vi "Test MQTT-3.1.2-12.vi"(8 "error in (no error)":errorcluster) -> (0 "error out":errorcluster)   [LabVIEW 2013]
uses:
  <vilib>/LabVIEW Open Source Project/MQTT Control Packets/Control Packets/ControlPacket/ControlPacket.lvclass
  <vilib>/LabVIEW Open Source Project/MQTT Control Packets/Control Packets/CONNECT/ConnectFlags -- cluster.ctl
  <vilib>/LabVIEW Open Source Project/MQTT Control Packets/Control Packets/ControlPacket/QualityOfService -- enum.ctl
  <vilib>/LabVIEW Open Source Project/MQTT Client/Client class/Client.lvclass/Client.ctl
  <vilib>/addons/_JKI Toolkits/Caraya/classes/Assert/Assert Equal Value_Variant.vi
  <vilib>/addons/_JKI Toolkits/Caraya/classes/Assert/Assert Equal Value and Type_Variant.vi
  <vilib>/LabVIEW Open Source Project/MQTT Control Packets/Control Packets/PUBLISH/PUBLISH.lvclass
  <vilib>/addons/_JKI Toolkits/Caraya/classes/Test/Test.lvclass
  <vilib>/addons/_JKI Toolkits/Caraya/classes/Assert/Assert.lvclass
  <vilib>/LabVIEW Open Source Project/MQTT Client/Client class/Client.lvclass
  <vilib>/LabVIEW Open Source Project/MQTT Connection/MQTT_Base/Base Class/MQTT_Base.lvclass
  <vilib>/LabVIEW Open Source Project/MQTT Control Packets/Control Packets/CONNECT/CONNECT.lvclass
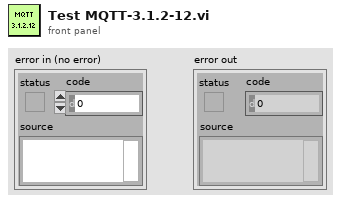
[diagram p1: front panel]
types:
  T1 = typedef "MQTT_Control_Packets.lvlib/ControlPacket.lvclass/QualityOfService -- enum.ctl" = enum16{"0 (At Most Once)", "1 (At Least Once)", "2 (Exactly Once)"}
  T2 = typedef "MQTT_Control_Packets.lvlib/CONNECT.lvclass/ConnectFlags -- cluster.ctl" = cluster{"Reserved":bool, "Clean Session":bool, "Will Flag":bool, "Will QoS 1":bool, "Will QoS 2":bool, "Will Retain":bool, "Password Flag":bool, "User Name Flag":bool}
  T3 = cluster{"Will Topic":string, "Will Message":string, "Username":string, "Password":string}
  T4 = typedef "MQTT Client.lvlib/Client.lvclass/Public Events -- cluster.ctl" = cluster{"Connection Status":refnum<user-event>, "Connected":refnum<user-event>, "Application Message":refnum<user-event>}
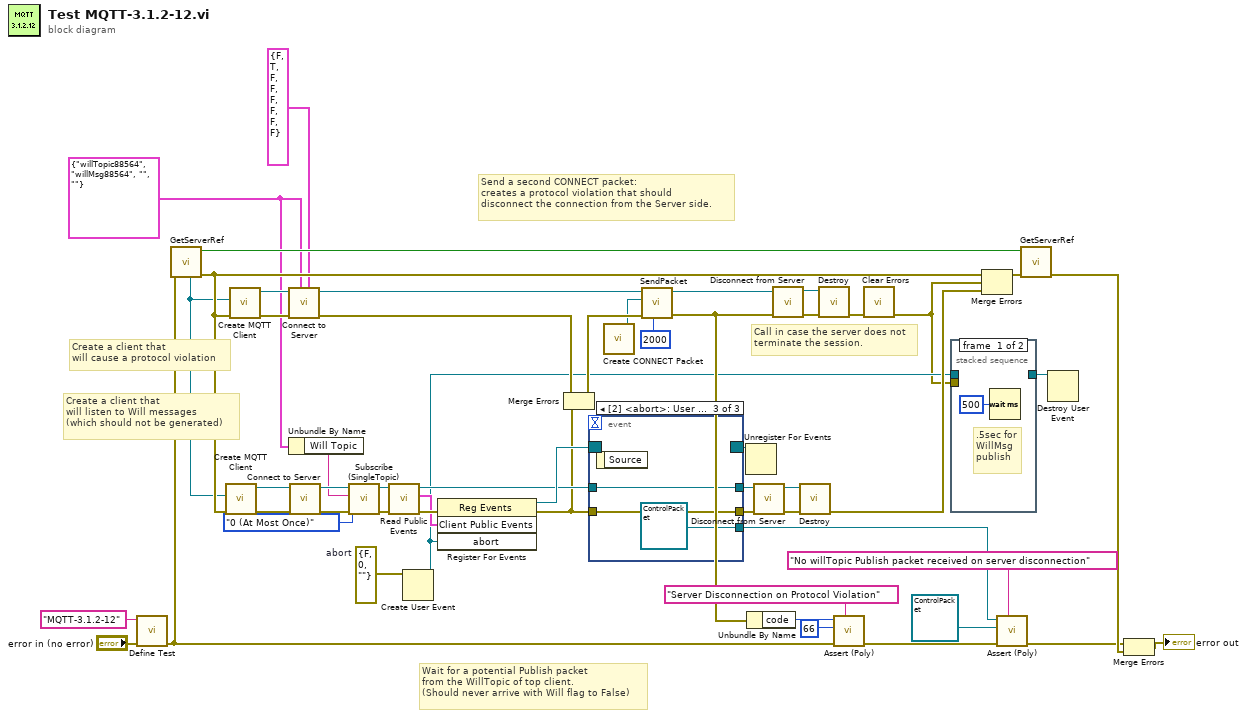
[diagram p0: block diagram]
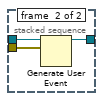
[diagram p2: hidden frame]
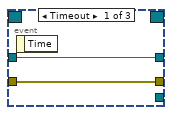
[diagram p3: hidden frame]
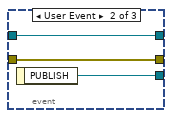
[diagram p4: hidden frame]
diagram:
  w20 = errorcluster {"status"=FALSE, "code"=0, "source"=""}  # abort
  w30 = T3 {"Will Topic"="willTopic88564", "Will Message"="willMsg88564", "Username"="", "Password"=""} ("Payload")
  # "Wait for a potential Publish packet\nfrom the WillTopic of top client.\n(Should never arrive with Will flag to False)"
  # "Create a client that\nwill listen to Will messages\n(which should not be generated)"
  # "Create a client that\nwill cause a protocol violation"
  # "Call in case the server does not\nterminate the session."
  # "Send a second CONNECT packet:\ncreates a protocol violation that should\ndisconnect the connection from the Server side."
  n1 = call <vilib>:"Define Test.vi"("error in (no error)"="error in (no error)", "Label (VI Title)"="MQTT-3.1.2-12") -> ("error out"=w48:errorcluster)  [unwired: 9 in]
  n2 = call "GetServerRef.vi"("error in"=w48) -> ("error out"=w34:errorcluster, "Created"=w49:bool, "Connection Config"=w1:refnum<class "Connection.lvclass">)  [unwired: 7 in, 1 out]
  n3 = call <vilib>:"Create MQTT Client.vi"("error in (no error)"=w34, "Connection Configuration"=w1) -> ("error out"=w33:errorcluster, "Client out"=w32:refnum<class "Client.lvclass">)  [unwired: 8 in]
  n4 = call <vilib>:"Create MQTT Client.vi"("error in (no error)"=w34, "Connection Configuration"=w1) -> ("error out"=w44:errorcluster, "Client out"=w45:refnum<class "Client.lvclass">)  [unwired: 8 in]
  n5 = call <vilib>:"Connect to Server.vi"("Connect Flags"=T2 {"Reserved"=FALSE, "Clean Session"=TRUE, "Will Flag"=FALSE, "Will QoS 1"=FALSE, "Will QoS 2"=FALSE, "Will Retain"=FALSE, "Password Flag"=FALSE, "User Name Flag"=FALSE}, "Payload"=w30, "error in (no error)"=w44, "Client in"=w45) -> ("error out"=w27:errorcluster, "Client out"=w43:refnum<class "Client.lvclass">)  [unwired: 4 in, 2 out]
  n6 = Unbundle By Name(w30) -> ("Will Topic"=w29:string)
  n7 = call <vilib>:"Connect to Server.vi"("error in (no error)"=w33, "Client in"=w32) -> ("error out"=w28:errorcluster, "Client out"=w31:refnum<class "Client.lvclass">)  [unwired: 6 in, 2 out]
  n8 = call <vilib>:"Subscribe (SingleTopic).vi"("error in (no error)"=w28, "QoS"=QualityOfService_--_enum."0 (At Most Once)", "Topic Filter"=w29, "MQTT_Base in"=w31) -> ("error out"=w24:errorcluster, "MQTT_Base out"=w25:refnum<class "Client.lvclass">)  [unwired: 5 in, 1 out]
  n9 = call <vilib>:"Read Public Events.vi"("error in (no error)"=w24, "Client in"=w25) -> ("error out"=w23:errorcluster, "Client Public Events"=w22:T4, "Client out"=w18:refnum<class "Client.lvclass">)  [unwired: 7 in]
  n10 = Create User Event(user event datatype=w20) -> (user event=w9:refnum<user-event>)  [unwired: 1 in, 1 out]
  n11 = register-events(error in=w23, w22, w9) -> (reference out=w21:refnum<event-registration>, error out=w17:errorcluster)  [unwired: 1 in]
  n12 = Merge Errors(w27, w17) -> (w26:errorcluster)
  n13 = event shown="[2] <abort>: User Event" {
    selector: w21 -> [_ _ _]
    dyn-events: [_ _ _] -> w19
    timeout: _ -> [_ _ _]
    tunnel: [_ w59 refnum<class "ControlPacket.lvclass"> refnum ("ControlPacket")] -> w10
    tunnel: w18 -> [w56 w58 w62]
    tunnel: w17 -> [w55 w57 w61]
    tunnel: [w56 w58 w62] -> w14
    tunnel: [w55 w57 w61] -> w13
    event Timeout {
      n14 = event-data() -> ()  [unwired: 1 in, 1 out]
    }
    event User Event {
      n15 = event-data() -> ("PUBLISH"=w59:refnum<class "PUBLISH.lvclass">)  [unwired: 1 in]
    }
    event User Event {
      n16 = event-data() -> ()  [unwired: 1 in, 1 out]
    }
  }
  n17 = call <vilib>:"Create CONNECT Packet.vi"() -> ("CONNECT"=w5:refnum<class "CONNECT.lvclass">)  [unwired: 9 in, 2 out]
  n18 = call <vilib>:"SendPacket.vi"("timeout (0ms : no ack)"=2000, "error in (no error)"=w26, "ControlPacket"=w5, "Client in"=w43) -> ("error out"=w37:errorcluster, "Client out"=w39:refnum<class "Client.lvclass">)  [unwired: 5 in, 1 out]
  n19 = Unregister For Events(event registration refnum=w19) -> ()  [unwired: 1 in, 1 out]
  n20 = Unbundle By Name(w37) -> ("code"=w46:i32)
  n21 = call <vilib>:"Disconnect from Server.vi"("error in (no error)"=w13, "Client in"=w14) -> ("error out"=w16:errorcluster, "Client out"=w15:refnum<class "Client.lvclass">)  [unwired: 7 in, 1 out]
  n22 = call <vilib>:"Disconnect from Server.vi"("error in (no error)"=w37, "Client in"=w39) -> ("error out"=w40:errorcluster, "Client out"=w41:refnum<class "Client.lvclass">)  [unwired: 7 in, 1 out]
  n23 = call <vilib>:"Destroy.vi"("error in (no error)"=w16, "MQTT_Base in"=w15) -> ("error out"=w12:errorcluster)  [unwired: 8 in, 1 out]
  n24 = call <vilib>:"Destroy.vi"("error in (no error)"=w40, "MQTT_Base in"=w41) -> ("error out"=w38:errorcluster)  [unwired: 8 in, 1 out]
  n25 = call-poly <vilib>:"Assert (Poly).vi"("Label"="Server Disconnection on Protocol Violation", "error in (no error)"=w48, "Y"=66 ("code"), "X"=w46) -> ("error out"=w36:errorcluster)  [unwired: 7 in]
  n26 = call <vilib>:"Clear Errors.vi"("error in (no error)"=w38) -> ("error out"=w8:errorcluster)  [unwired: 6 in]
  n27 = stacked-sequence {
    tunnel: w9 -> [_ w66]
    tunnel: w8 -> [_ w65]
    tunnel: [_ w64] -> w7
    frame #0 {
      # ".5sec for\nWillMsg\npublish"
      n28 = Wait (ms)(milliseconds to wait=u32 500) -> ()  [unwired: 1 out]
    }
    frame #1 {
      n29 = Generate User Event(user event=w66, event data cluster=w65) -> (user event out=w64:refnum<user-event>)  [unwired: 2 in, 1 out]
    }
  }
  n30 = Merge Errors(w34, w8, w12) -> (w11:errorcluster)
  n31 = call-poly <vilib>:"Assert (Poly).vi"("Label"="No willTopic Publish packet received on server disconnection", "error in (no error)"=w36, "Y"=refnum<class "ControlPacket.lvclass"> refnum ("ControlPacket"), "X"=w10) -> ("error out"=w35:errorcluster)  [unwired: 7 in]
  n32 = call "GetServerRef.vi"("error in"=w11, "Destroy (F)"=w49) -> ("error out"=w47:errorcluster)  [unwired: 6 in, 3 out]
  n33 = Destroy User Event(user event=w7) -> ()  [unwired: 1 in, 1 out]
  n34 = Merge Errors(w35, w47) -> (→"error out":errorcluster)
